vi "CE Client - Close session.vi"(6 "error in":errorcluster, 9 "CE session":T1={"VI refnum"=refnum, "VC Handle"=-1}) -> (0 "error out":errorcluster, 3 "CE session out":T1={"VI refnum"=refnum, "VC Handle"=-1})   [LabVIEW 2021]
doc: "::: CalcExpress Toolkit :::\nCopyright (c) 2000-2026 Konstantin Shifershteyn. All rights reserved."
uses:
  CE Session.ctl
  vi.lib/addons/CalcExpress/cetypes.llb/VarMan Variable Context Handle.ctl
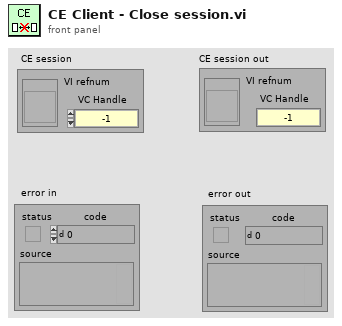
[diagram p1: front panel]
types:
  T1 = typedef "CE Session.ctl" = cluster{"VI refnum":refnum<vi>, "VC Handle":T2}
  T2 = typedef "VarMan Variable Context Handle.ctl" = i32
  T3 = enum16{"open session", "close session", "CalcExpress", "VarMan", "VarMan (low level)"}
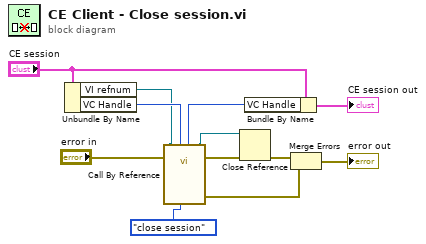
[diagram p0: block diagram]
diagram:
  n1 = Unbundle By Name("CE session") -> ("VI refnum"=w4:refnum<vi>, "VC Handle"=w11:T2)
  n2 = call-by-ref "?"(reference=w4, error in="error in", "exec"=T3."close session", "VC Handle"=w11) -> (reference out=w10:refnum<vi>, error out=w8:errorcluster, "error out"=w2:errorcluster, "VC Handle out"=w7:i32)  [unwired: 7 in, 1 out]
  n3 = Close Reference(reference=w10, error in (no error)=w8) -> (error out=w3:errorcluster)
  n4 = Bundle By Name(cluster="CE session", "VC Handle"=w7) -> (→"CE session out":T1)
  n5 = Merge Errors(w3, w2) -> (→"error out":errorcluster)
